vi "Draw.vi"(8 "error in (no error)":errorcluster, 10 "2D Picture in":picture, 11 "Picture in":refnum<class "Image.lvclass">) -> (0 "error out":errorcluster, 2 "2D Picture out":picture, 3 "Picture out":refnum<class "Image.lvclass">)   [LabVIEW 2021, in "Picture2D.lvlib" / "Image.lvclass"]
uses:
  Image.lvclass
  PointSpecialized/PointSpecialized.lvclass
  C:/GitHub/Picture2D/src/Point/Point.lvclass
  ColorRGBA/ColorRGBA.lvclass
  PointSpecialized/PointSpecialized.lvclass/PointSpecialized.ctl
  PointSpecialized/GetColor.vi
  Point/Point.lvclass
  Color/Color.lvclass
  Picture2D/Picture2D.lvlib
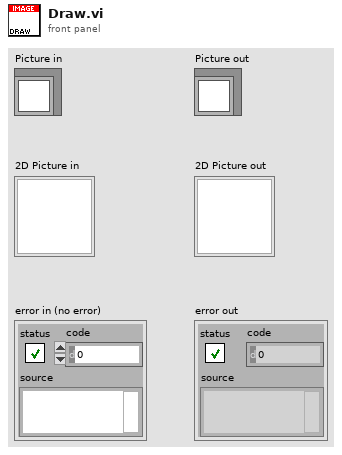
[diagram p1: front panel]
types:
  T1 = typedef "imagedata.ctl" = cluster{"image type":i32, "image depth":i32, "image":u8[], "mask":u8[], "colors":u32[], "Rectangle":cluster{"left":i16, "top":i16, "right":i16, "bottom":i16}}
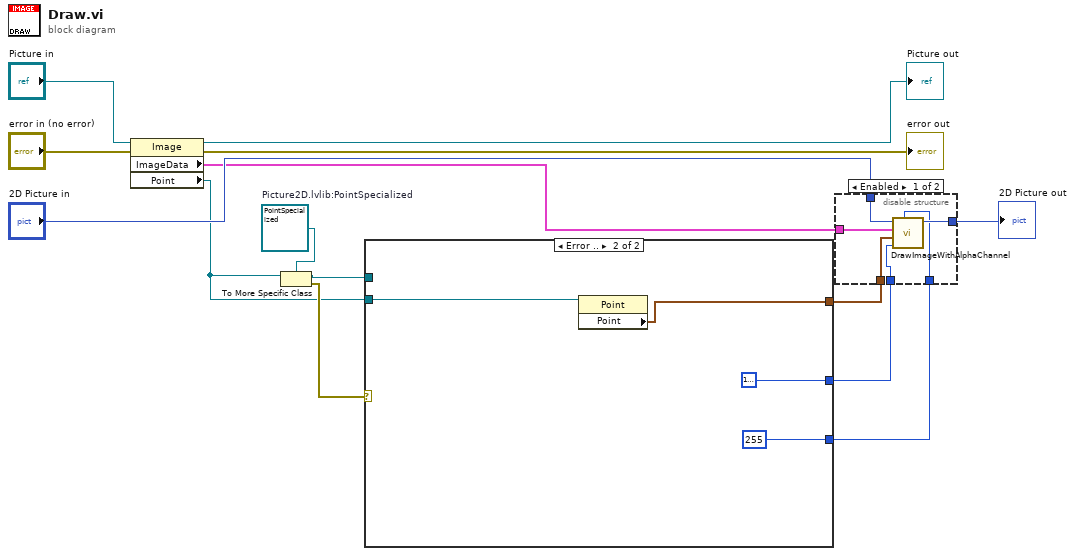
[diagram p0: block diagram]
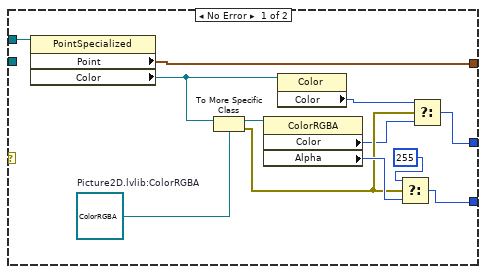
[diagram p2: hidden frame]
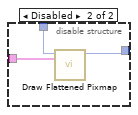
[diagram p3: hidden frame]
diagram:
  w7 = refnum<class "PointSpecialized.lvclass"> refnum  # Picture2D.lvlib:PointSpecialized
  n1 = property class="Image"(reference="Picture in", error in="error in (no error)") -> (reference out=→"Picture out":refnum<class "Image.lvclass">, error out=→"error out":errorcluster, "ImageData"=w8:T1, "Point"=w1:refnum<class "Point.lvclass">)
  n2 = To More Specific Class(target class=w7, reference=w1) -> (specific class reference=w6:refnum<class "PointSpecialized.lvclass">, error out=w3:errorcluster)  [unwired: 1 in]
  n3 = case shown="Error .." w3 {
    tunnel: w6 -> [w26 _]
    tunnel: [w25 w27] -> w5
    tunnel: [w15 u32 16777216 ("Color")] -> w4
    tunnel: [w21 u8 255 ("Alpha")] -> w2
    tunnel: w1 -> [_ w28]
    frame No Error {
      w23 = refnum<class "ColorRGBA.lvclass"> refnum  # Picture2D.lvlib:ColorRGBA
      n4 = property class="PointSpecialized"(reference=w26) -> ("Point"=w25:cluster{"x":i16, "y":i16}, "Color"=w18:refnum<class "Color.lvclass">)  [unwired: 1 in, 2 out]
      n5 = To More Specific Class(target class=w23, reference=w18) -> (specific class reference=w24:refnum<class "ColorRGBA.lvclass">, error out=w19:errorcluster)  [unwired: 1 in]
      n6 = property class="ColorRGBA"(reference=w24) -> ("Color"=w16:u32, "Alpha"=w22:u8)  [unwired: 1 in, 2 out]
      n7 = property class="Color"(reference=w18) -> ("Color"=w17:u32)  [unwired: 1 in, 2 out]
      n8 = Select(t=u8 255, s=w19, f=w22) -> (s? t:f=w21:u8)
      n9 = Select(t=w17, s=w19, f=w16) -> (s? t:f=w15:u32)
    }
    frame Error {
      n10 = property class="Point"(reference=w28) -> ("Point"=w27:cluster{"x":i16, "y":i16})  [unwired: 1 in, 2 out]
    }
  }
  n11 = disable-structure shown="Enabled" {
    disable-tunnel: w8 -> [w36 w37]
    disable-tunnel: "2D Picture in" -> [w35 w39]
    disable-tunnel: [w34 w38] -> w9
    disable-tunnel: w5 -> [w33 _]
    disable-tunnel: w4 -> [w32 _]
    disable-tunnel: w2 -> [w31 _]
    frame Enabled {
      n12 = call "DrawImageWithAlphaChannel.vi"("Alpha (255 opaque)"=w31, "Background Color"=w32, "Insertion Point(x,y)"=w33, "image data"=w36, "2D Picture in"=w35) -> ("2D Picture out"=w34:picture)  [unwired: 6 in]
    }
    frame Disabled {
      n13 = call <vilib>:"Draw Flattened Pixmap.vi"("image data"=w37, "picture"=w39) -> ("new picture"=w38:picture)  [unwired: 7 in]
    }
  }
  "2D Picture out" <- w9
